vi "ClassNode_Create.vi"(0 "reference":refnum<class "ClassNode.lvclass">, 5 "error in (no error)":errorcluster) -> (14 "reference out":refnum<class "ClassNode.lvclass">, 19 "error out":errorcluster)   [LabVIEW 2020, in "ClassNode.lvclass"]
doc: "Creates and initializes a new ClassNode object.\n\nThis object should be destroyed using a ClassNode destructor VI or a virtual base class destructor VI.\n\n[GOOP 2.1]"
uses:
  <resource>/Framework/Providers/Open_GDS/UML/ClassNode_class/ClassNode.lvclass
  C:/Program Files (x86)/National Instruments/LabVIEW 2020/resource/Framework/Providers/Open_GDS/UML/RectangularNode_class/RectangularNode.lvclass
  <resource>/Framework/Providers/Open_GDS/UML/MultiLineString_class/SizeType.ctl
  <resource>/Framework/Providers/Open_GDS/UML/MultiLineString_class/JustificationType.ctl
  <resource>/Framework/Providers/Open_GDS/UML/General/Rectangle/Rectangle Rectangle2D.ctl
  <resource>/Framework/Providers/Open_GDS/UML/RectangularNode_class/RectangularNode.lvclass
  <resource>/Framework/Providers/Open_GDS/UML/MultiLineString_class/MultiLineString.lvclass
panel:
  # "The input reference should only\nbe wired when this method is called\nby a sub class constructor."
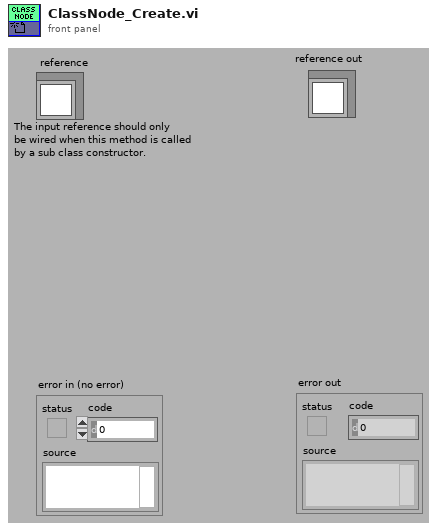
[diagram p1: front panel]
types:
  T1 = typedef "Rectangle Rectangle2D.ctl" = cluster{"x":dbl, "y":dbl, "width":dbl, "height":dbl}
  T2 = typedef "MultiLineString.lvclass/SizeType.ctl" = enum16{"LARGE", "NORMAL", "SMALL"}
  T3 = typedef "MultiLineString.lvclass/JustificationType.ctl" = enum16{"LEFT", "CENTER", "RIGHT"}
  T4 = typedef "ClassNode.lvclass/ObjectAttributes.ctl" = cluster{"midHeight":dbl, "botHeight":dbl, "name":refnum<class "MultiLineString.lvclass">, "attributes":refnum<class "MultiLineString.lvclass">, "methods":refnum<class "MultiLineString.lvclass">, "DEFAULT_COMPARTMENT_HEIGHT":i32, "DEFAULT_WIDTH":i32, "DEFAULT_HEIGHT":i32, "showMethods":bool, "showAttributes":bool, "ClassPath":path}
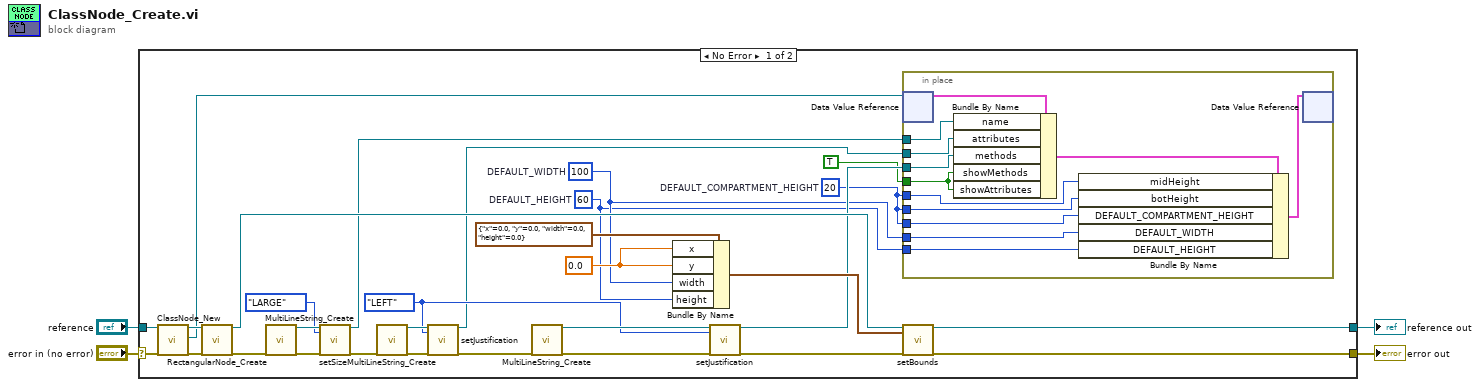
[diagram p0: block diagram]
diagram:
  n1 = case shown="No Error" "error in (no error)" {
    selector: "error in (no error)" -> [w34 w48]
    tunnel: [w6 w47] -> w4
    tunnel: [w5 w48] -> w3
    tunnel: "reference" -> [w33 w47]
    frame No Error {
      w16 = 0.0 ("x")
      w20 = JustificationType."LEFT" ("justification")
      w8 = 60  # DEFAULT_HEIGHT
      w9 = 100  # DEFAULT_WIDTH
      w10 = 20  # DEFAULT_COMPARTMENT_HEIGHT
      n2 = call <resource>:"ClassNode_New.vi"("reference in"=w33, "error in (no error)"=w34) -> ("reference out"=w31:refnum<class "ClassNode.lvclass">, "DVRRefOut"=w7:refnum<data-value>, "error out"=w32:errorcluster)  [unwired: 2 in, 13 out]
      n3 = call <resource>:"RectangularNode_Create.vi"("reference"=w31, "error in (no error)"=w32) -> ("reference out"=w19:refnum<class "ClassNode.lvclass">, "error out"=w30:errorcluster)  [unwired: 1 in, 15 out]
      n4 = call <resource>:"MultiLineString_Create.vi"("error in (no error)"=w30) -> ("reference out"=w25:refnum<class "MultiLineString.lvclass">, "error out"=w24:errorcluster)  [unwired: 2 in, 15 out]
      n5 = call <resource>:"setSize.vi"("reference"=w25, "size"=SizeType."LARGE", "error in (no error)"=w24) -> ("reference out"=w14:refnum<class "MultiLineString.lvclass">, "error out"=w23:errorcluster)  [unwired: 15 out]
      n6 = call <resource>:"MultiLineString_Create.vi"("error in (no error)"=w23) -> ("reference out"=w29:refnum<class "MultiLineString.lvclass">, "error out"=w28:errorcluster)  [unwired: 2 in, 15 out]
      n7 = call <resource>:"setJustification.vi"("reference"=w29, "justification"=w20, "error in (no error)"=w28) -> ("reference out"=w13:refnum<class "MultiLineString.lvclass">, "error out"=w22:errorcluster)  [unwired: 15 out]
      n8 = call <resource>:"MultiLineString_Create.vi"("error in (no error)"=w22) -> ("reference out"=w27:refnum<class "MultiLineString.lvclass">, "error out"=w26:errorcluster)  [unwired: 2 in, 15 out]
      n9 = Bundle By Name(cluster=T1 {"x"=0.0, "y"=0.0, "width"=0.0, "height"=0.0} ("bounds"), "x"=w16, "y"=w16, "width"=w9, "height"=w8) -> (w18:T1)
      n10 = call <resource>:"setJustification.vi"("reference"=w27, "justification"=w20, "error in (no error)"=w26) -> ("reference out"=w12:refnum<class "MultiLineString.lvclass">, "error out"=w15:errorcluster)  [unwired: 15 out]
      n11 = in-place {
        in-place-border: w14 -> [w45]
        in-place-border: w13 -> [w44]
        in-place-border: w12 -> [w43]
        in-place-border: TRUE ("showMethods") -> [w42]
        in-place-border: w10 -> [w40]
        in-place-border: w10 -> [w39]
        in-place-border: w10 -> [w38]
        in-place-border: w9 -> [w37]
        in-place-border: w8 -> [w36]
        n12 = in-place-dvr #1(w7) -> (w46:T4)  [unwired: 1 out]
        n13 = Bundle By Name(cluster=w46, "name"=w45, "attributes"=w44, "methods"=w43, "showMethods"=w42, "showAttributes"=w42) -> (w41:T4)
        n14 = Bundle By Name(cluster=w41, "midHeight"=w40, "botHeight"=w39, "DEFAULT_COMPARTMENT_HEIGHT"=w38, "DEFAULT_WIDTH"=w37, "DEFAULT_HEIGHT"=w36) -> (w35:T4)
        n15 = in-place-dvr #1(w35) -> ()  [unwired: 2 out]
      }
      n16 = call-dynamic "setBounds.vi"("reference"=w19, "bounds"=w18, "error in (no error)"=w15) -> ("reference out"=w6:refnum<class "ClassNode.lvclass">, "error out"=w5:errorcluster)  [unwired: 15 in]
    }
    frame Error {
    }
  }
  "error out" <- w3
  "reference out" <- w4
